vi "Zero AO Outputs.vi"(8 "error in (no error)":errorcluster, 9 "channels":i32[](array[numeric]), 10 "zero":T1, 11 "Instrument.DAQ in":refnum<class "Instrument.DAQ.lvclass">) -> (0 "error out":errorcluster, 1 "Saved Offsets":dbl[](array[numeric]), 2 "Saved Amplitudes":dbl[](array[numeric]), 3 "Instrument.DAQ out":refnum<class "Instrument.DAQ.lvclass">)   [LabVIEW 2019, in "Instrument.Lockin.lvlib" / "Instrument.DAQ.lvclass"]
uses:
  Instrument.DAQ.lvclass
  Lockin.Typedefs/API/Lockin.measureInputOffset.zero--enum.ctl
  Instrument.DAQ.lvclass/Instrument.DAQ.ctl
  Lockin.Typedefs/Lockin.Typedefs.lvlib
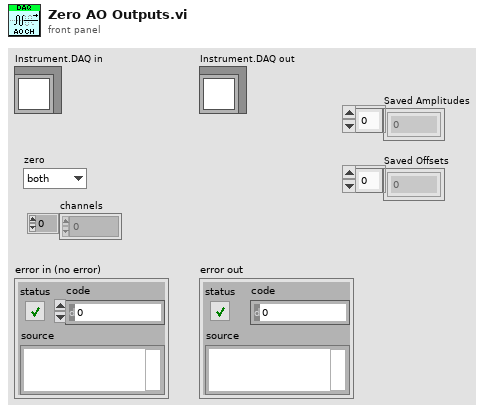
[diagram p1: front panel]
types:
  T1 = typedef "Lockin.Typedefs.lvlib/Lockin.measureInputOffset.zero--enum.ctl" = enum16{"both", "ac", "dc", "none"}
  T2 = typedef "Lockin.Typedefs.lvlib/AO.Channel--Cluster--Array.ctl" = T3[]
  T3 = typedef "Lockin.Typedefs.lvlib/AO.Channel--Cluster.ctl" = cluster{"Enable?":bool, "Channel":i32, "Amplitude":dbl, "Offset":dbl, "Frequency":dbl, "Phase":dbl, "Function":T4, "Sweeping?":bool, "Limit AC":bool, "Limit DC?":bool, "Duty Cycle":bool}
  T4 = typedef "Lockin.Typedefs.lvlib/AO.Channel.Function--Enum.ctl" = enum16{"sine", "square", "triangle", "saw"}
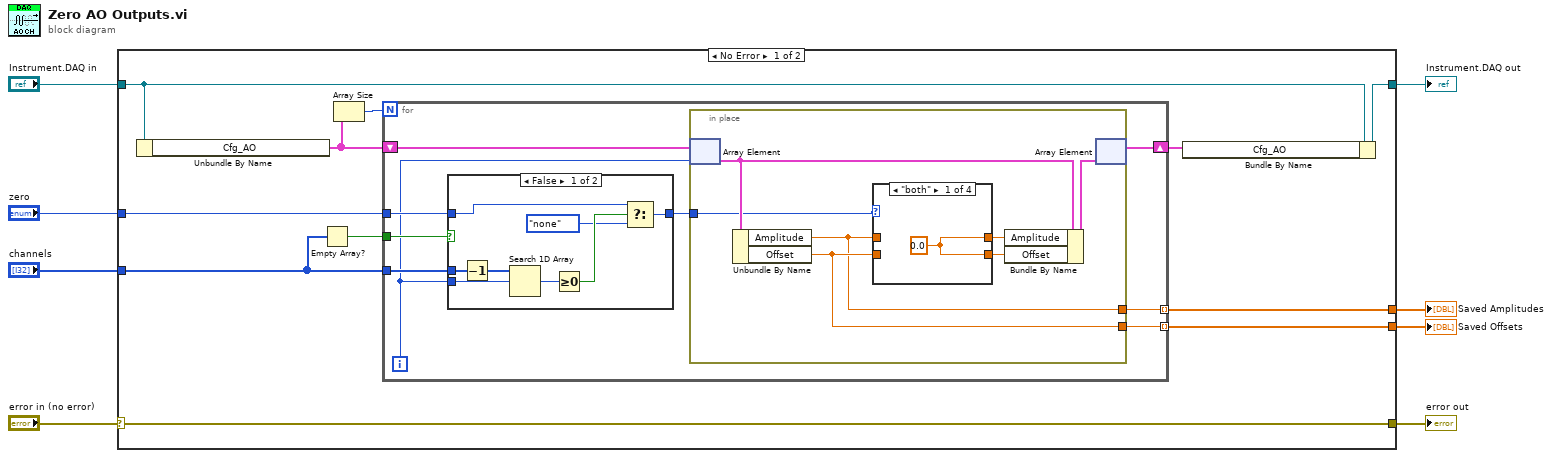
[diagram p0: block diagram]
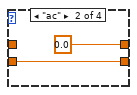
[diagram p3: hidden frame]
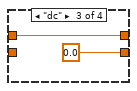
[diagram p4: hidden frame]
diagram:
  n1 = case shown="No Error" "error in (no error)" {
    selector: "error in (no error)" -> [w14 w53]
    tunnel: [w18 w52] -> w8
    tunnel: "Instrument.DAQ in" -> [w17 w52]
    tunnel: [w15 _] -> w6
    tunnel: [w14 w53] -> w4
    tunnel: [w13 _] -> w3
    tunnel: "zero" -> [w12 _]
    tunnel: "channels" -> [w11 _]
    frame No Error {
      n2 = Unbundle By Name(w17) -> ("Cfg_AO"=w16:T2)
      n3 = Empty Array?(array=w11) -> (empty?=w9:bool)
      n4 = Array Size(array=w16) -> (size(s)=w10:i32)
      n5 = for {
        N: w10 -> [_]
        tunnel: [w28] -> w15 mode=indexing
        shift-right: [w26] -> w19
        shift-left: w16 -> [w27]
        tunnel: [w25] -> w13 mode=indexing
        tunnel: w12 -> [w22]
        tunnel: w11 -> [w21]
        tunnel: w9 -> [w24]
        i -> [w20]
        n6 = case shown="False" w24 {
          tunnel: [w31 w37] -> w23
          tunnel: w22 -> [w30 w37]
          tunnel: w21 -> [w36 _]
          tunnel: w20 -> [w34 _]
          frame False {
            n7 = Decrement(x=w36) -> (x-1=w35:i32[])
            n8 = Search 1D Array(1D array=w35, element=w34) -> (index of element=w33:i32)  [unwired: 1 in]
            n9 = Greater Or Equal To 0?(x=w33) -> (x >= 0?=w32:bool)
            n10 = Select(t=w30, s=w32, f=Lockin.measureInputOffset.zero--enum."none" ("t")) -> (s? t:f=w31:T1)
          }
          frame True {
          }
        }
        n11 = in-place {
          in-place-border: [w38] -> w28
          in-place-border: [w39] -> w25
          in-place-border: w23 -> [w42]
          n12 = in-place-array #1(w27, w20) -> (w44:T3)
          n13 = Unbundle By Name(w44) -> ("Amplitude"=w38:dbl, "Offset"=w39:dbl)
          n14 = case shown="\"both\"" w42 {
            tunnel: [w45 0.0 ("Amplitude") w48 w51] -> w41
            tunnel: [w45 w46 0.0 ("Offset") w50] -> w40
            tunnel: w39 -> [_ w46 _ w50]
            tunnel: w38 -> [_ _ w48 w51]
            frame "both" {
              w45 = 0.0 ("Amplitude")
            }
            frame "ac" {
            }
            frame "dc" {
            }
            frame "none", Default {
            }
          }
          n15 = Bundle By Name(cluster=w44, "Amplitude"=w41, "Offset"=w40) -> (w43:T3)
          n16 = in-place-array #1(w43) -> (w26:T2)  [unwired: 1 out]
        }
      }
      n17 = Bundle By Name(cluster=w17, "Cfg_AO"=w19) -> (w18:refnum<class "Instrument.DAQ.lvclass">)
    }
    frame Error {
    }
  }
  "error out" <- w4
  "Instrument.DAQ out" <- w8
  "Saved Amplitudes" <- w6
  "Saved Offsets" <- w3
